vi "Measurement Logic.vi"() -> ()   [LabVIEW 2021, in "NIFgenStandardFunction.lvlib"]
uses:
  NIFgenStandardFunction.lvlib
  Measurement Results.ctl
  <vilib>/Plug-In SDKs/Clients/Session Management V1/Session Reservation/Session Reservation.lvclass
  <vilib>/Plug-In SDKs/Measurements/Measure Call Context/Measure Call Context.lvclass
  <vilib>/Plug-In SDKs/Sessions/niFGEN/NI Session Management niFGEN.lvlib
  Measurement Configuration.ctl
  Waveform.ctl
panel:
  out "measure call context out":refnum<class "Measure Call Context.lvclass">
  in  "measure call context in":refnum<class "Measure Call Context.lvclass">
  out "measurement results":T1={"actual_duration"=1.0}
  in  "measurement configuration":T2={"pin_name"="", "waveform"=enum."Noise", "frequency"=6.0, "amplitude"=6.0, "duration"=6.0}
  out "error out":errorcluster
  in  "error in":errorcluster
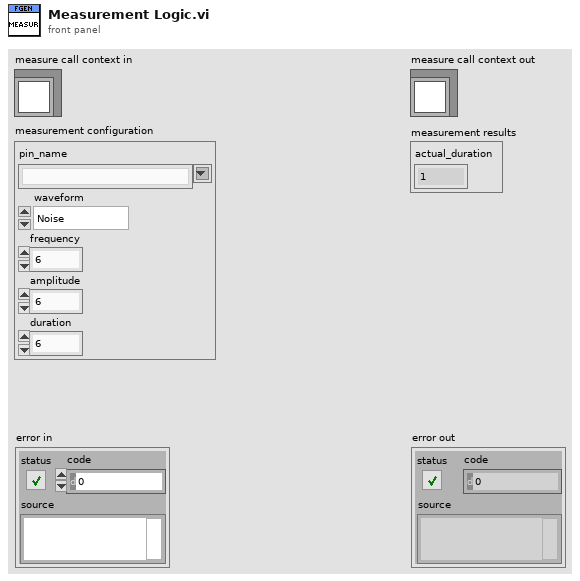
[diagram p1: front panel]
types:
  T1 = typedef "NIFgenStandardFunction.lvlib/Measurement Results.ctl" = cluster{"actual_duration":dbl}
  T2 = typedef "NIFgenStandardFunction.lvlib/Measurement Configuration.ctl" = cluster{"pin_name":string, "waveform":T3, "frequency":dbl, "amplitude":dbl, "duration":dbl}
  T3 = typedef "NIFgenStandardFunction.lvlib/Waveform.ctl" = enum32{"Sine", "Square", "Triangle", "Ramp Up", "Ramp Down", "DC", "Noise", "User"}
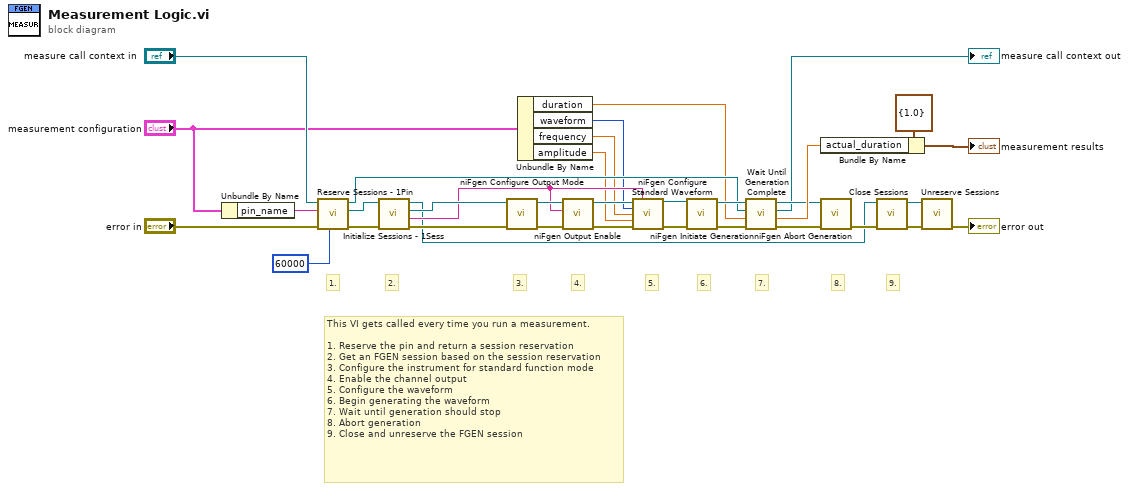
[diagram p0: block diagram]
diagram:
  # "9."
  # "8."
  # "7."
  # "6."
  # "5."
  # "4."
  # "3."
  # "2."
  # "This VI gets called every time you run a measurement.\n\n1. Reserve the pin and return a session reservation\n2. Get an FGEN session based on the session reservation\n3. Configure the instrument for standard function mode\n4. Enable the channel output\n5. Configure the waveform\n6. Begin generating the waveform\n7. Wait until generation should stop\n8. Abort generation\n9. Close and unreserve the FGEN session"
  # "1."
  n1 = Unbundle By Name("measurement configuration") -> ("pin_name"=w33:string)
  n2 = call <vilib>:"Reserve Sessions - 1Pin.vi"("timeout (ms)"=60000, "error in"="error in", "pin or relay name"=w33, "measurement context in"="measure call context in") -> ("error out"=w31:errorcluster, "session reservation out"=w30:refnum<class "Session Reservation.lvclass">, "measurement context out"=w7:refnum<class "Measure Call Context.lvclass">)  [unwired: 5 in]
  n3 = call <vilib>:"Initialize Sessions - 1Sess.vi"("error in"=w31, "session reservation in"=w30) -> ("error out"=w15:errorcluster, "channel list"=w12:string, "session"=w14:refnum<k15>, "session reservation out"=w10:refnum<class "Session Reservation.lvclass">)  [unwired: 6 in]
  n4 = call <instrlib>:"niFgen Configure Output Mode.vi"("error in (no error)"=w15, "Instrument Handle"=w14) -> ("error out"=w24:errorcluster, "Instrument Handle Out"=w25:refnum<k15>)  [unwired: 7 in]
  n5 = Unbundle By Name("measurement configuration") -> ("duration"=w1:dbl, "waveform"=w2:T3, "frequency"=w3:dbl, "amplitude"=w4:dbl)
  n6 = call <instrlib>:"niFgen Output Enable.vi"("error in (no error)"=w24, "Channel Name"=w12, "Instrument Handle"=w25) -> ("error out"=w23:errorcluster, "Instrument Handle Out"=w22:refnum<k15>)  [unwired: 7 in]
  n7 = call <instrlib>:"niFgen Configure Standard Waveform.vi"("Instrument Handle"=w22, "Channel Name"=w12, "Waveform"=w2, "Frequency"=w3, "Amplitude"=w4, "error in (no error)"=w23) -> ("Instrument Handle Out"=w21:refnum<k15>, "error out"=w20:errorcluster)  [unwired: 8 in]
  n8 = call <instrlib>:"niFgen Initiate Generation.vi"("error in (no error)"=w20, "Instrument Handle"=w21) -> ("error out"=w19:errorcluster, "Instrument Handle Out"=w8:refnum<k15>)  [unwired: 8 in]
  n9 = call "Wait Until Generation Complete.vi"("error in"=w19, "duration"=w1, "measurement context in"=w7, "instrument handle in"=w8) -> ("error out"=w18:errorcluster, "actual duration"=w16:dbl, "measurement context out"=→"measure call context out":refnum<class "Measure Call Context.lvclass">, "instrument handle out"=w6:refnum<k15>)  [unwired: 4 in]
  n10 = Bundle By Name(cluster=T1 {"actual_duration"=1.0} ("measurement results"), "actual_duration"=w16) -> (→"measurement results":T1)
  n11 = call <instrlib>:"niFgen Abort Generation.vi"("error in (no error)"=w18, "Instrument Handle"=w6) -> ("error out"=w11:errorcluster)  [unwired: 8 in, 1 out]
  n12 = call <vilib>:"Close Sessions.vi"("error in"=w11, "session reservation in"=w10) -> ("error out"=w28:errorcluster, "session reservation out"=w27:refnum<class "Session Reservation.lvclass">)  [unwired: 8 in]
  n13 = call <vilib>:"Unreserve Sessions.vi"("error in"=w28, "session reservation in"=w27) -> ("error out"=→"error out":errorcluster)  [unwired: 9 in]
